vi "read_key_integer.vi"(7 "table":string, 8 "error in (no error)":errorcluster, 9 "default (0)":i64, 10 "key":string, 11 "toml in":refnum<class "toml.lvclass">) -> (0 "error out":errorcluster, 1 "value":i64, 3 "toml out":refnum<class "toml.lvclass">)   [LabVIEW 2020, in "toml.lvclass"]
uses:
  toml.lvclass
  Doc/Doc.lvclass
  Table/Table.lvclass
  0e0b1f61-b1d6-4a7f-b7e8-bf687aa3a0f4.vi
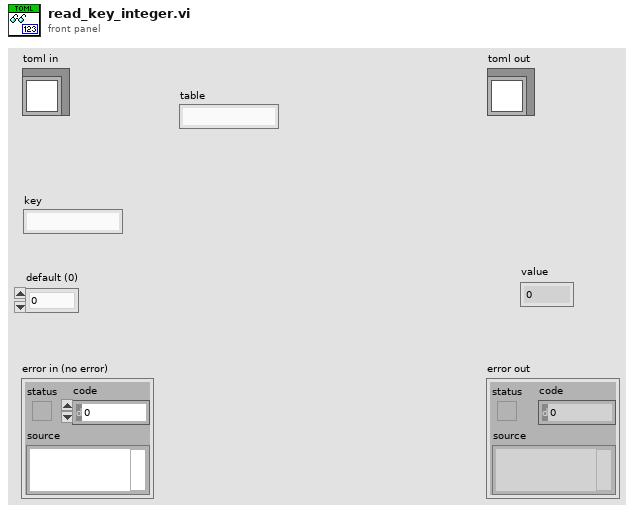
[diagram p1: front panel]
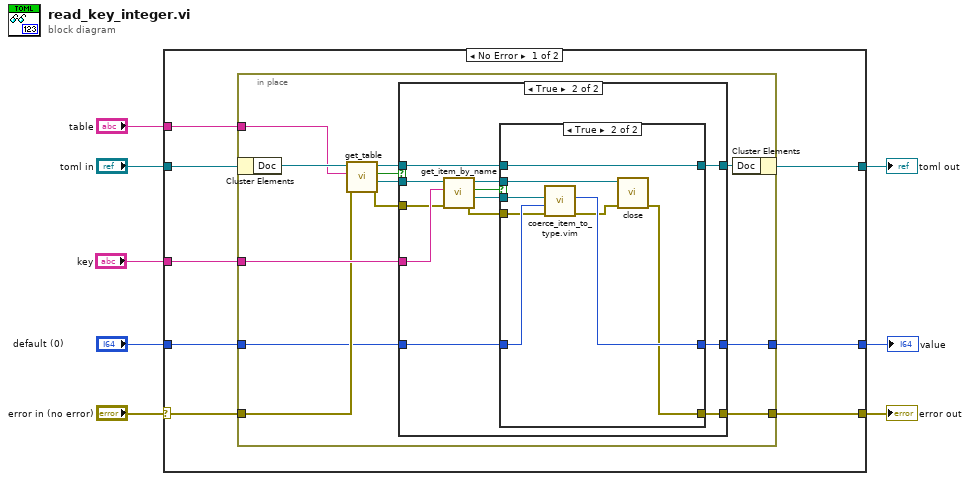
[diagram p0: block diagram]
diagram:
  n1 = case shown="No Error" "error in (no error)" {
    selector: "error in (no error)" -> [w10 w56]
    tunnel: [w11 w56] -> w7
    tunnel: [w15 w55] -> w5
    tunnel: "toml in" -> [w16 w55]
    tunnel: "table" -> [w14 _]
    tunnel: "key" -> [w13 _]
    tunnel: "default (0)" -> [w12 _]
    tunnel: [w9 _] -> w1
    frame No Error {
      n2 = in-place {
        in-place-border: w14 -> [w21]
        in-place-border: w13 -> [w24]
        in-place-border: w12 -> [w19]
        in-place-border: [w23] -> w11
        in-place-border: w10 -> [w22]
        in-place-border: [w18] -> w9
        n3 = in-place-cluster #1(w16) -> ("Doc"=w26:refnum<class "Doc.lvclass">)
        n4 = call "get_table.vi"("error in (no error)"=w22, "table_name"=w21, "Doc in"=w26) -> ("error out"=w20:errorcluster, "Table"=w28:refnum<class "Table.lvclass">, "found?"=w17:bool, "Doc out"=w27:refnum<class "Doc.lvclass">)  [unwired: 5 in]
        n5 = case shown="True" w17 {
          tunnel: w28 -> [_ w43]
          tunnel: w27 -> [w31 w42]
          tunnel: [w31 w40] -> w25
          tunnel: w24 -> [_ w39]
          tunnel: [w29 w38] -> w23
          tunnel: w20 -> [w29 w37]
          tunnel: w19 -> [w30 w35]
          tunnel: [w30 w34] -> w18
          frame False {
          }
          frame True {
            n6 = call "get_item_by_name.vi"("error in (no error)"=w37, "item_name"=w39, "Table in"=w43) -> ("error out"=w33:errorcluster, "Item"=w36:refnum<class "Item.lvclass">, "found?"=w32:bool, "Table out"=w41:refnum<class "Table.lvclass">)  [unwired: 4 in, 1 out]
            n7 = case shown="True" w32 {
              tunnel: w42 -> [w44 w54]
              tunnel: w41 -> [_ w49]
              tunnel: [w44 w54] -> w40
              tunnel: [w45 w47] -> w38
              tunnel: w36 -> [_ w53]
              tunnel: w35 -> [w46 w52]
              tunnel: [w46 w51] -> w34
              tunnel: w33 -> [w45 w50]
              frame False {
              }
              frame True {
                n8 = call "coerce_item_to_type.vim"("error in (no error)"=w50, "default (\"\")"=w52, "Item in"=w53) -> ("error out"=w48:errorcluster, "value"=w51:i64)  [unwired: 7 in]
                n9 = call "close.vi"("error in (no error)"=w48, "Table in"=w49) -> ("error out"=w47:errorcluster)  [unwired: 9 in]
              }
            }
          }
        }
        n10 = in-place-cluster #1("Doc"=w25) -> (w15:refnum<class "toml.lvclass">)
      }
    }
    frame Error {
    }
  }
  "error out" <- w7
  "toml out" <- w5
  "value" <- w1
